vi "DQMH_Get All IDs.vi"(0 "Module 1":string, 1 "Module 2":string, 2 "Module 3":string, 3 "Module 4":string, 4 "Module 5":string, 5 "Module 6":string, 6 "Modules":T1, 7 "error in":errorcluster) -> (13 "error out":errorcluster, 14 "Module 1":i32, 15 "Module 2":i32, 16 "Module 3":i32, 17 "Module 4":i32, 18 "Module 5":i32, 19 "Module 6":i32)   [LabVIEW 2025, in "Sequencer.lvlib"]
uses:
  Libraries/Sequencer/Sequencer.lvlib
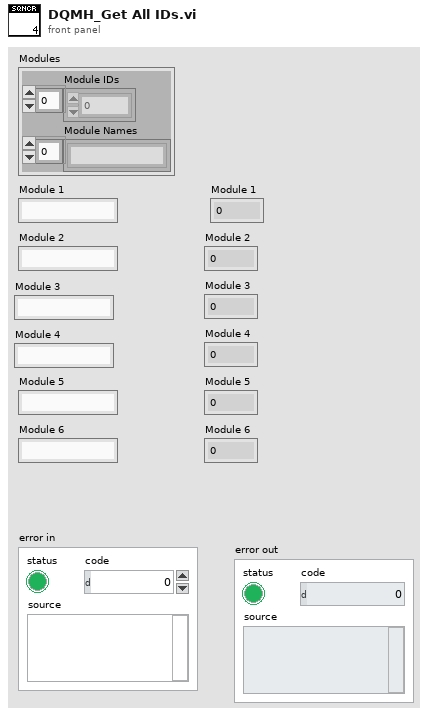
[diagram p1: front panel]
types:
  T1 = cluster{"Module IDs":i32[], "Module Names":string[]}
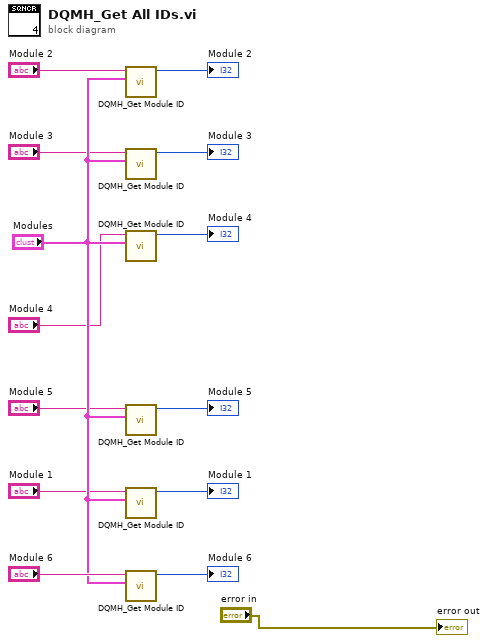
[diagram p0: block diagram]
diagram:
  n1 = call "DQMH_Get Module ID.vi"("Modules"="Modules", "Module Name"="Module 2") -> ("Module ID out"=→"Module 2":i32)  [unwired: 9 in]
  n2 = call "DQMH_Get Module ID.vi"("Modules"="Modules", "Module Name"="Module 3") -> ("Module ID out"=→"Module 3":i32)  [unwired: 9 in]
  n3 = call "DQMH_Get Module ID.vi"("Modules"="Modules", "Module Name"="Module 4") -> ("Module ID out"=→"Module 4":i32)  [unwired: 9 in]
  n4 = call "DQMH_Get Module ID.vi"("Modules"="Modules", "Module Name"="Module 5") -> ("Module ID out"=→"Module 5":i32)  [unwired: 9 in]
  n5 = call "DQMH_Get Module ID.vi"("Modules"="Modules", "Module Name"="Module 1") -> ("Module ID out"=→"Module 1":i32)  [unwired: 9 in]
  n6 = call "DQMH_Get Module ID.vi"("Modules"="Modules", "Module Name"="Module 6") -> ("Module ID out"=→"Module 6":i32)  [unwired: 9 in]
  "error out" <- "error in"
